vi "test--Mixed.vi"(11 "Test Case In":refnum<class "Hex to Color.lvclass">) -> (0 "error out":errorcluster, 3 "Test Case Out":refnum<class "Hex to Color.lvclass">)   [LabVIEW 2021, in "Hex to Color.lvclass"]
uses:
  Hex to Color.lvclass
  C:/Program Files/National Instruments/LabVIEW 2024/vi.lib/Astemes/LUnit/Test Case.lvclass
  <vilib>/Astemes/LUnit/Test Case.lvclass/Test Case.ctl
  4993e8ee-a06a-463a-9684-69129f64d5ce.vi
  src/Material SubVIs/tsc--RGB to Color.vi
  <vilib>/Astemes/LUnit/Core/LUnit Test Case/Private/Append Pass Result.vi
  <vilib>/Astemes/LUnit/Core/LUnit Test Case/Private/Append Fail Result.vi
  4993e8ee-a06a-463a-9684-69129f64d5ce.vi/9c5d11cd-9439-4240-a1ee-d9baace9c924.vi
  <vilib>/Astemes/LUnit/Core/LUnit Test Case/Private/Run In UI.vi
  <vilib>/Utility/error.llb/Clear Errors.vi
  src/Material SubVIs/Material SubVIs.lvlib
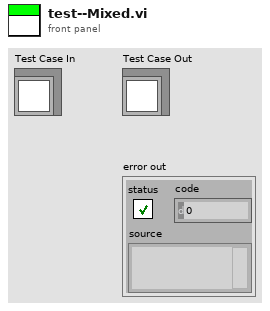
[diagram p1: front panel]
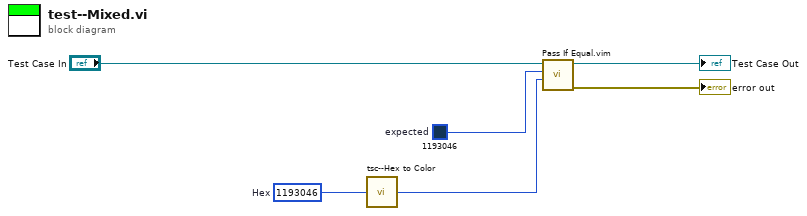
[diagram p0: block diagram]
diagram:
  w1 = u32 1193046  # expected
  w3 = u32 1193046  # Hex
  n1 = call "tsc--Hex to Color.vi"("Hex String"=w3) -> ("Color"=w2:u32)  [unwired: 4 in]
  n2 = call "Pass If Equal.vim"("Actual"=w2, "Expected"=w1, "LUnit Test Case In"="Test Case In") -> ("error out"=→"error out":errorcluster, "LUnit Test Case Out"=→"Test Case Out":refnum<class "Hex to Color.lvclass">)  [unwired: 7 in]
